vi "Get Status.vi"(8 "error in":errorcluster, 11 "UI GUID":string) -> (0 "error out":errorcluster, 3 "Messages":i32)   [LabVIEW 2025, in "CAN-LIN Raw Bus Capture UI.lvlib"]
uses:
  CAN-LIN Raw Bus Capture UI.lvlib
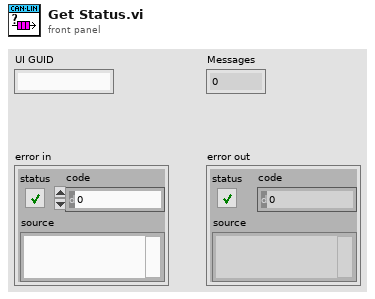
[diagram p1: front panel]
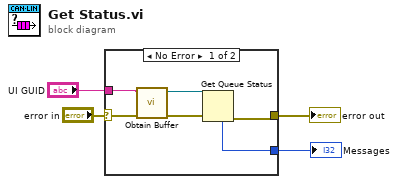
[diagram p0: block diagram]
diagram:
  n1 = case shown="No Error" "error in" {
    selector: "error in" -> [w6 w11]
    tunnel: [w10 w11] -> w3
    tunnel: [w9 _] -> w2
    tunnel: "UI GUID" -> [w5 _]
    frame No Error {
      n2 = call "Obtain Buffer.vi"("error in (no error)"=w6, "UI GUID"=w5) -> ("error out"=w8:errorcluster, "Table Queue"=w7:refnum<queue>)  [unwired: 8 in]
      n3 = Get Queue Status(queue=w7, error in (no error)=w8) -> (error out=w10:errorcluster, # elements in queue=w9:i32)  [unwired: 1 in, 6 out]
    }
    frame Error {
    }
  }
  "error out" <- w3
  "Messages" <- w2
